vi "Generate AO Sweep Waveforms.vi"(8 "error in (no error)":errorcluster, 11 "Generator":refnum<class "Generator.lvclass">) -> (0 "error out":errorcluster, 2 "AO Array":waveform(dbl)[](array[waveform]), 3 "Generator out":refnum<class "Generator.lvclass">)   [LabVIEW 2019, in "Generator.lvclass"]
uses:
  Generator.lvclass
  typedefs/Generator.Sweep Status--enum.ctl
  typedefs/Generator.Sweep State--enum.ctl
  Generator.lvclass/Generator.ctl
  Waveform.Attributes/Waveform.Attributes.lvlib
panel:
  in  "Tab Control":enum32{"Page 1", "Graphs"}(tab)
  out "Waveform Graph":waveform(dbl)[](graph)
  out "sweep status":T1
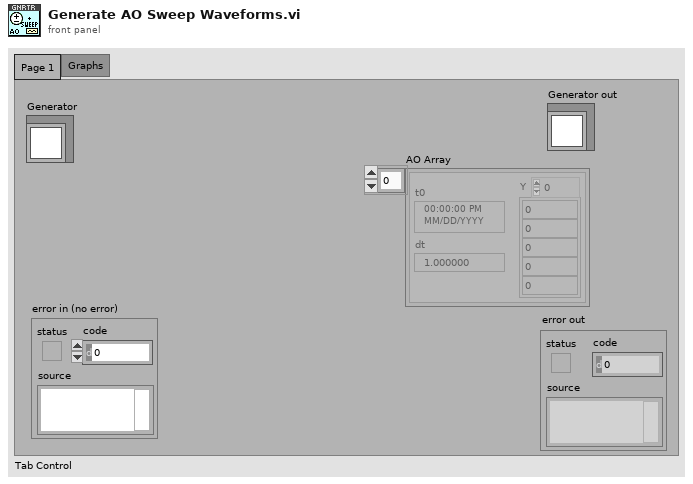
[diagram p1: front panel]
types:
  T1 = typedef "Generator.lvclass/Generator.Sweep Status--enum.ctl" = enum16{"idle", "initializing", "waiting", "sweeping", "stopping"}
  T2 = typedef "Generator.lvclass/Generator.Sweep State--enum.ctl" = enum16{"idle", "initialize", "wait", "sweep", "stop"}
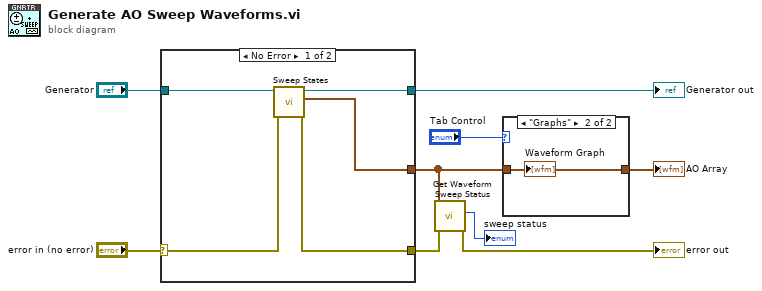
[diagram p0: block diagram]
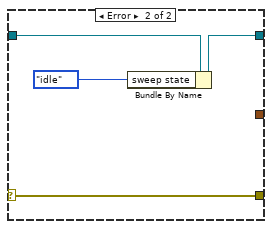
[diagram p2: hidden frame]
diagram:
  n1 = case shown="No Error" "error in (no error)" {
    selector: "error in (no error)" -> [w11 w18]
    tunnel: "Generator" -> [w14 w15]
    tunnel: [w13 w16] -> w8
    tunnel: [w12 w18] -> w3
    tunnel: [w10 _] -> w4
    frame No Error {
      n2 = call "Sweep States.vi"("error in (no error)"=w11, "Generator in"=w14) -> ("error out"=w12:errorcluster, "Waveforms out"=w10:waveform(dbl)[], "Generator out"=w13:refnum<class "Generator.lvclass">)  [unwired: 7 in]
    }
    frame Error {
      n3 = Bundle By Name(cluster=w15, "sweep state"=Generator.Sweep_State--enum."idle" ("sweep state out")) -> (w16:refnum<class "Generator.lvclass">)
    }
  }
  "Generator out" <- w8
  n4 = call "Get Waveform Sweep Status.vi"("error in (no error)"=w3, "Waveforms in"=w4) -> ("error out"=→"error out":errorcluster, "sweep status"=→"sweep status":T1)  [unwired: 7 in, 1 out]
  n5 = case shown="\"Graphs\"" "Tab Control" {
    tunnel: w4 -> [w19 w20]
    tunnel: [w19 w20] -> w5
    frame Default {
    }
    frame "Graphs" {
      "Waveform Graph" <- w20
    }
  }
  "AO Array" <- w5
